vi "validate line configuration.vi"(7 "EthernetIP configuration":refnum<class "EIP Tags Configuration.lvclass">, 11 "line in":T1) -> (1 "valid?":bool, 2 "problem":string, 3 "line out":T1)   [LabVIEW 2013, in "EIP Tags editor node.lvclass"]
uses:
  EIP Tags editor node.lvclass
  table line.ctl
  channel/EIP Tags Channel.lvclass
  configuration/EIP Tags Configuration.lvclass
  <vilib>/NI/Tag Bus/tag/Data Type.ctl
  <vilib>/NI/Tag Bus/tag/tag descriptor.lvclass/tag descriptor.ctl
  channel/EIP Tags Channel.lvclass/EIP Tags Channel.ctl
  configuration/EIP Tags Configuration.lvclass/EIP Tags Configuration.ctl
  configuration/read eip channels.vi
  configuration/Read EIP tags.vi
  <vilib>/NI/Tag Bus/tag/read tag name.vi
  channel/Read EIP Tag UUID.vi
  channel/Read element.vi
  <vilib>/NI/Tag Bus/tag/read data type.vi
  <vilib>/NI/Tag Bus/tag/tag descriptor.lvclass
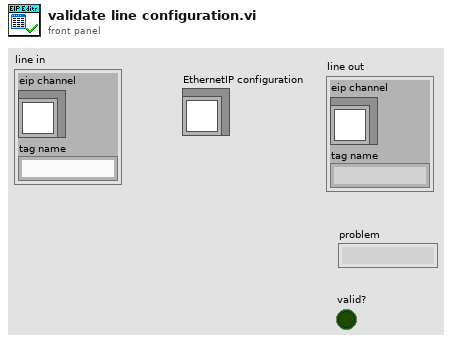
[diagram p1: front panel]
types:
  T1 = typedef "EIP Tags editor node.lvclass/table line.ctl" = cluster{"eip channel":refnum<class "EIP Tags Channel.lvclass">, "tag name":string}
  T2 = typedef "tag bus.lvlib/tag descriptor.lvclass/Data Type.ctl" = enum16{"Double", "Single", "I64", "I32", "I16", "I8", "U64", "U32", "U16", "U8", "Boolean", "String", "Array of Double", "Array of Single", "Array of I64", "Array of I32", "Array of I16", "Array of I8", "Array of U64", "Array of U32", "Array of U16", "Array of U8", "Array of Boolean", "Array of String"}
  T3 = typedef "EIP Tags Configuration.lvclass/eip tag definition.ctl" = cluster{"eip tag types":T4, "unique tag name":string, "Number of Elements":u32}
  T4 = typedef "EIP Tags Configuration.lvclass/eip tag types.ctl" = enum16{"SINT", "INT", "DINT", "REAL", "BOOL", "STRING"}
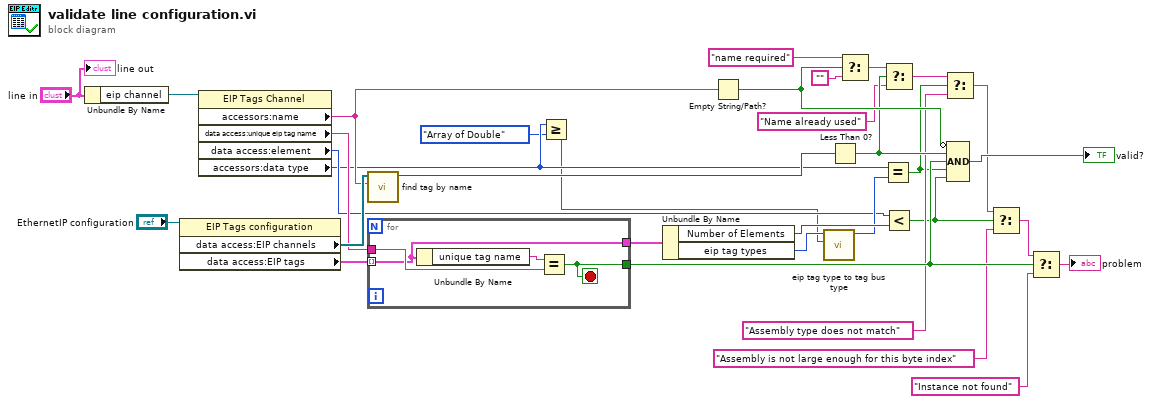
[diagram p0: block diagram]
diagram:
  n1 = Unbundle By Name("line in") -> ("eip channel"=w32:refnum<class "EIP Tags Channel.lvclass">)
  n2 = property class="EIP Tags configuration"(reference="EthernetIP configuration") -> ("data access:EIP channels"=w30:refnum<class "EIP Tags Channel.lvclass">[], "data access:EIP tags"=w26:T3[])  [unwired: 1 in, 2 out]
  n3 = property class="EIP Tags Channel"(reference=w32) -> ("accessors:name"=w29:string, "data access:unique eip tag name"=w20:string, "data access:element"=w4:i32, "accessors:data type"=w3:T2)  [unwired: 1 in, 2 out]
  n4 = call <vilib>:"find tag by name.vi"("name"=w29, "tags in"=w30) -> ("index"=w27:i32)  [unwired: 9 in]
  n5 = for {
    tunnel: w26 -> [w35] mode=indexing
    tunnel: w20 -> [w36]
    tunnel: [w35] -> w14
    tunnel: [w34] -> w18
    stop <- w34 stop-if-true
    n6 = Unbundle By Name(w35) -> ("unique tag name"=w37:string)
    n7 = Equal?(x=w37, y=w36) -> (x = y?=w34:bool)
  }
  n8 = Greater Or Equal?(x=w3, y=Data_Type."Array of Double") -> (x >= y?=w1:bool)
  n9 = Unbundle By Name(w14) -> ("Number of Elements"=w9:u32, "eip tag types"=w6:T4)
  n10 = Empty String/Path?(string/path=w29) -> (empty?=w25:bool)
  n11 = call "eip tag type to tag bus type.vi"("array?"=w1, "eip tag types"=w6) -> ("data type"=w5:T2)  [unwired: 9 in]
  n12 = Less Than 0?(x=w27) -> (x < 0?=w24:bool)
  n13 = Select(t="name required", s=w25, f="") -> (s? t:f=w23:string)
  n14 = Equal?(x=w3, y=w5) -> (x = y?=w10:bool)
  n15 = Select(t=w23, s=w24, f="Name already used") -> (s? t:f=w13:string)
  n16 = Less?(x=w4, y=w9) -> (x < y?=w8:bool)
  n17 = Select(t=w13, s=w10, f="Assembly type does not match") -> (s? t:f=w15:string)
  n18 = Compound Arithmetic op=AND(invert w25, w24, w18, w10, w8) -> (→"valid?":bool)
  n19 = Select(t=w15, s=w8, f="Assembly is not large enough for this byte index") -> (s? t:f=w12:string)
  n20 = Select(t=w12, s=w18, f="Instance not found") -> (s? t:f=→"problem":string)
  "line out" <- "line in"
